vi "2021-07-09.vi"() -> ()   [LabVIEW 2019]
panel:
  out "time":cluster{i32[], i32[]}[](graph)
  out "throughput":cluster{i32[], dbl[]}[](graph)
  out "message rate":cluster{i32[], dbl[]}[](graph)
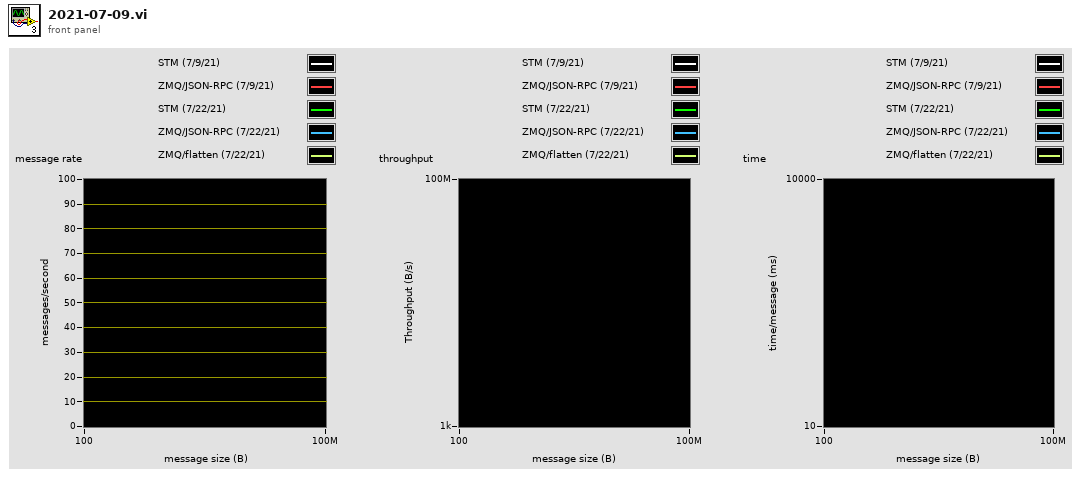
[diagram p1: front panel]
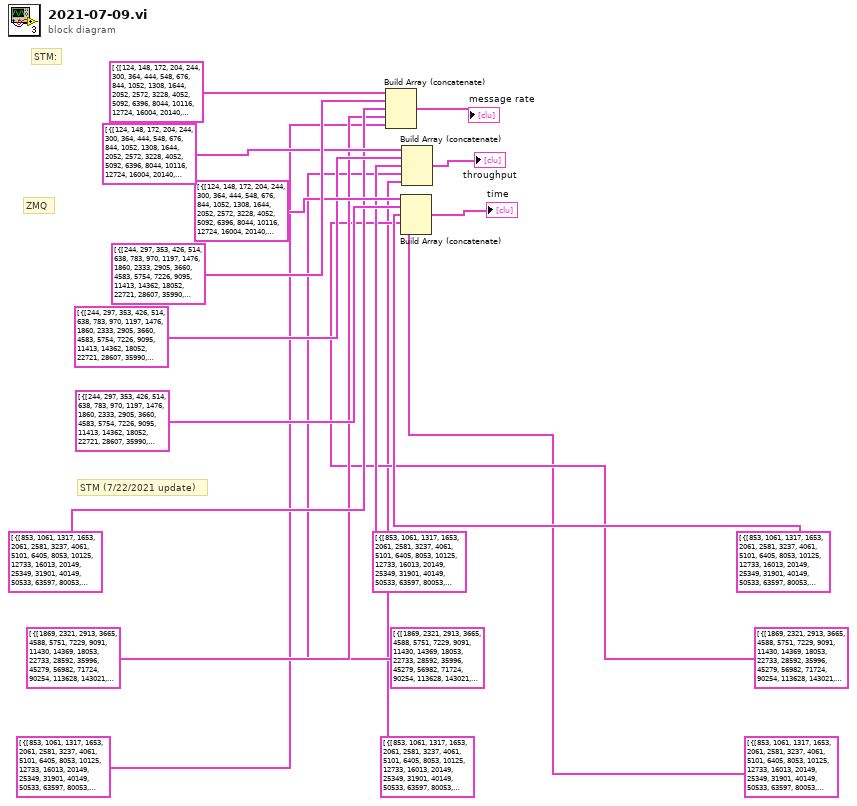
[diagram p0: block diagram]
diagram:
  # "STM (7/22/2021 update)"
  # "ZMQ"
  # "STM:"
  n1 = Build Array (concatenate)(cluster{i32[], dbl[]}[] [{[124, 148, 172, 204, 244, 300, 364, 444, 548, 676, 844, 1052, 1308, 1644, 2052, 2572, 3228, 4052, 5092, 6396, 8044, 10116, 12724, 16004, 20140, 25340, 31892, 40140, 50524, 63588, 80044, 100756, 126836, 159668, 200996, 253028, 318532, 400996, 504812, 635508, 800044, 1007188, 1267956, 1596252, 2009556, 2529868, 3184900, 4009540, 5047700, 6354668, 8000044], [73.26007326007326, 37.31343283582089, 80.32128514056225, 80.97165991902834, 83.68200836820084, 81.30081300813008, 81.30081300813008, 81.30081300813008, 80.0, 81.9672131147541, 82.3045267489712, 82.98755186721992, 81.30081300813008, 82.98755186721992, 82.3045267489712, 80.64516129032258, 80.97165991902834, 81.9672131147541, 82.64462809917356, 82.64462809917356, 81.63265306122449, 80.0, 81.9672131147541, 82.64462809917356, 78.43137254901961, 82.3045267489712, 81.30081300813008, 80.64516129032258, 80.0, 80.0, 79.6812749003984, 79.6812749003984, 79.6812749003984, 75.18796992481202, 77.22007722007721, 74.07407407407408, 71.94244604316546, 69.68641114982579, 66.22516556291392, 62.30529595015576, 57.636887608069166, 50.125313283208015, 36.03603603603603, 31.84713375796178, 27.06359945872801, 23.80952380952381, 18.099547511312217, 13.89854065323141, 9.47867298578199, 7.163323782234958, 5.396654074473826]}] ("message rate"), cluster{i32[], dbl[]}[] [{[244, 297, 353, 426, 514, 638, 783, 970, 1197, 1476, 1860, 2333, 2905, 3660, 4583, 5754, 7226, 9095, 11413, 14362, 18052, 22721, 28607, 35990, 45262, 57027, 71748, 90267, 113711, 142986, 180100, 226656, 285362, 359078, 452157, 569307, 716716, 902172, 1135653, 1430011, 1799736, 2265809, 2852633, 3591256, 4521510, 5691835, 7165085, 9020945, 11356828, 14298020, 17999563], [60.42296072507553, 60.6060606060606, 60.6060606060606, 62.5, 63.09148264984227, 58.139534883720934, 65.359477124183, 68.4931506849315, 54.200542005420054, 62.11180124223603, 60.06006006006006, 65.78947368421053, 63.291139240506325, 51.41388174807198, 63.492063492063494, 64.1025641025641, 56.81818181818182, 65.14657980456026, 56.81818181818182, 54.94505494505495, 50.76142131979695, 49.26108374384236, 50.25125628140703, 49.75124378109452, 51.0204081632653, 44.54342984409799, 42.918454935622314, 40.48582995951417, 39.920159680638726, 37.38317757009346, 32.62642740619902, 28.40909090909091, 24.96878901373283, 21.141649048625794, 18.18181818181818, 14.388489208633095, 12.453300124533001, 10.655301012253597, 8.003201280512204, 6.736274840013473, 5.442176870748299, 4.519774011299435, 3.7064492216456637, 2.983738624496494, 2.384358607534573, 1.9719976336028398, 1.5360983102918588, 1.238927089140804, 0.963762528912876, 0.7363228039172374, 0.598623166716552]}] ("message rate 2"), cluster{i32[], dbl[]}[] [{[853, 1061, 1317, 1653, 2061, 2581, 3237, 4061, 5101, 6405, 8053, 10125, 12733, 16013, 20149, 25349, 31901, 40149, 50533, 63597, 80053, 100765, 126845, 159677, 201005, 253037, 318541, 401005, 504821, 635517, 800053, 1007197, 1267965, 1596261, 2009565, 2529877, 3184909, 4009549, 5047709, 6354677, 8000053], [86.58008658008657, 87.33624454148472, 84.03361344537815, 85.47008547008546, 85.83690987124463, 85.47008547008546, 84.74576271186442, 85.83690987124463, 86.58008658008657, 86.20689655172413, 85.83690987124463, 85.1063829787234, 85.1063829787234, 84.74576271186442, 85.47008547008546, 86.20689655172413, 85.83690987124463, 85.1063829787234, 84.03361344537815, 82.3045267489712, 81.9672131147541, 82.64462809917356, 82.3045267489712, 80.64516129032258, 80.32128514056225, 79.6812749003984, 78.125, 74.07407407407408, 68.72852233676976, 69.68641114982579, 66.44518272425249, 59.347181008902076, 47.16981132075472, 39.920159680638726, 29.806259314456035, 26.52519893899204, 21.62162162162162, 16.142050040355123, 11.46131805157593, 9.7799511002445, 8.012820512820513]}] ("message rate"), cluster{i32[], dbl[]}[] [{[1869, 2321, 2913, 3665, 4588, 5751, 7229, 9091, 11430, 14369, 18053, 22733, 28592, 35996, 45279, 56982, 71724, 90254, 113628, 143021, 179910, 226633, 285458, 359226, 452070, 569242, 716757, 902238, 1135863, 1429968, 1799833, 2266041, 2852441, 3591671, 4520575, 5692223], [48.07692307692308, 95.23809523809524, 82.98755186721992, 88.88888888888889, 86.58008658008657, 81.63265306122449, 81.30081300813008, 79.05138339920948, 78.74015748031496, 74.9063670411985, 72.46376811594202, 70.92198581560284, 68.25938566552901, 64.72491909385113, 59.52380952380952, 56.980056980056986, 52.770448548812666, 45.04504504504504, 55.71030640668524, 42.19409282700422, 30.627871362940276, 32.520325203252035, 24.301336573511545, 19.821605550049554, 17.574692442882252, 13.812154696132596, 11.031439602868174, 8.92458723784025, 6.715916722632639, 5.303632988597189, 4.039587962027873, 3.2997855139415937, 2.839698991906858, 2.18435998252512, 1.7462673535318258, 1.3844662882458811]}] ("message rate"), cluster{i32[], dbl[]}[] [{[853, 1061, 1317, 1653, 2061, 2581, 3237, 4061, 5101, 6405, 8053, 10125, 12733, 16013, 20149, 25349, 31901, 40149, 50533, 63597, 80053, 100765, 126845, 159677, 201005, 253037, 318541, 401005, 504821, 635517, 800053, 1007197, 1267965, 1596261, 2009565, 2529877, 3184909, 4009549, 5047709, 6354677, 8000053], [78.125, 79.6812749003984, 77.82101167315174, 78.74015748031496, 81.30081300813008, 79.6812749003984, 79.6812749003984, 79.05138339920948, 79.36507936507937, 80.0, 77.82101167315174, 80.0, 79.05138339920948, 78.74015748031496, 80.0, 79.6812749003984, 78.125, 78.125, 78.43137254901961, 78.125, 77.22007722007721, 76.33587786259541, 76.62835249042145, 76.04562737642586, 72.992700729927, 71.17437722419928, 67.79661016949153, 64.72491909385113, 59.88023952095808, 56.17977528089888, 50.63291139240506, 43.47826086956522, 30.2571860816944, 26.917900403768506, 22.988505747126435, 20.876826722338205, 17.74622892635315, 14.673514306676449, 11.641443538998836, 9.775171065493646, 7.760962359332558]}] ("message rate")) -> (→"message rate":cluster{i32[], dbl[]}[])
  n2 = Build Array (concatenate)(cluster{i32[], i32[]}[] [{[124, 148, 172, 204, 244, 300, 364, 444, 548, 676, 844, 1052, 1308, 1644, 2052, 2572, 3228, 4052, 5092, 6396, 8044, 10116, 12724, 16004, 20140, 25340, 31892, 40140, 50524, 63588, 80044, 100756, 126836, 159668, 200996, 253028, 318532, 400996, 504812, 635508, 800044, 1007188, 1267956, 1596252, 2009556, 2529868, 3184900, 4009540, 5047700, 6354668, 8000044], [14, 27, 12, 12, 12, 12, 12, 12, 12, 12, 12, 12, 12, 12, 12, 12, 12, 12, 12, 12, 12, 12, 12, 12, 13, 12, 12, 12, 12, 12, 13, 13, 13, 13, 13, 14, 14, 14, 15, 16, 17, 19, 27, 31, 36, 41, 54, 71, 104, 138, 183]}] ("time"), cluster{i32[], i32[]}[] [{[244, 297, 353, 426, 514, 638, 783, 970, 1197, 1476, 1860, 2333, 2905, 3660, 4583, 5754, 7226, 9095, 11413, 14362, 18052, 22721, 28607, 35990, 45262, 57027, 71748, 90267, 113711, 142986, 180100, 226656, 285362, 359078, 452157, 569307, 716716, 902172, 1135653, 1430011, 1799736, 2265809, 2852633, 3591256, 4521510, 5691835, 7165085, 9020945, 11356828, 14298020, 17999563], [17, 16, 16, 16, 16, 17, 15, 15, 18, 16, 17, 15, 16, 19, 16, 16, 18, 15, 18, 18, 20, 20, 20, 20, 20, 22, 23, 25, 25, 27, 31, 35, 40, 47, 55, 70, 80, 94, 125, 148, 183, 221, 269, 335, 418, 506, 650, 805, 1035, 1355, 1666]}] ("time 2"), cluster{i32[], i32[]}[] [{[853, 1061, 1317, 1653, 2061, 2581, 3237, 4061, 5101, 6405, 8053, 10125, 12733, 16013, 20149, 25349, 31901, 40149, 50533, 63597, 80053, 100765, 126845, 159677, 201005, 253037, 318541, 401005, 504821, 635517, 800053, 1007197, 1267965, 1596261, 2009565, 2529877, 3184909, 4009549, 5047709, 6354677, 8000053], [12, 11, 12, 12, 12, 12, 12, 12, 11, 12, 12, 12, 12, 12, 12, 12, 12, 12, 12, 12, 12, 12, 12, 12, 12, 12, 12, 13, 14, 14, 14, 16, 20, 24, 32, 36, 44, 58, 83, 97, 119]}] ("time"), cluster{i32[], i32[]}[] [{[1869, 2321, 2913, 3665, 4588, 5751, 7229, 9091, 11430, 14369, 18053, 22733, 28592, 35996, 45279, 56982, 71724, 90254, 113628, 143021, 179910, 226633, 285458, 359226, 452070, 569242, 716757, 902238, 1135863, 1429968, 1799833, 2266041, 2852441, 3591671, 4520575, 5692223], [21, 10, 12, 11, 12, 12, 12, 13, 13, 13, 14, 14, 15, 15, 17, 18, 19, 22, 18, 24, 33, 31, 41, 50, 57, 72, 90, 112, 149, 188, 247, 302, 351, 457, 572, 721]}] ("time"), cluster{i32[], i32[]}[] [{[853, 1061, 1317, 1653, 2061, 2581, 3237, 4061, 5101, 6405, 8053, 10125, 12733, 16013, 20149, 25349, 31901, 40149, 50533, 63597, 80053, 100765, 126845, 159677, 201005, 253037, 318541, 401005, 504821, 635517, 800053, 1007197, 1267965, 1596261, 2009565, 2529877, 3184909, 4009549, 5047709, 6354677, 8000053], [13, 12, 13, 13, 12, 13, 13, 13, 13, 12, 13, 12, 13, 13, 12, 12, 13, 13, 13, 13, 13, 13, 13, 13, 13, 14, 14, 15, 16, 17, 19, 22, 32, 36, 42, 46, 54, 65, 82, 98, 122]}] ("time")) -> (→"time":cluster{i32[], i32[]}[])
  n3 = Build Array (concatenate)(cluster{i32[], dbl[]}[] [{[124, 148, 172, 204, 244, 300, 364, 444, 548, 676, 844, 1052, 1308, 1644, 2052, 2572, 3228, 4052, 5092, 6396, 8044, 10116, 12724, 16004, 20140, 25340, 31892, 40140, 50524, 63588, 80044, 100756, 126836, 159668, 200996, 253028, 318532, 400996, 504812, 635508, 800044, 1007188, 1267956, 1596252, 2009556, 2529868, 3184900, 4009540, 5047700, 6354668, 8000044], [9084.249084249084, 5522.388059701492, 13815.261044176706, 16518.218623481782, 20418.410041841005, 24390.243902439026, 29593.49593495935, 36097.560975609755, 43840.0, 55409.83606557377, 69465.02057613169, 87302.90456431535, 106341.46341463414, 136431.53526970954, 168888.8888888889, 207419.35483870967, 261376.51821862347, 332131.1475409836, 420826.4462809918, 528595.0413223141, 656653.0612244898, 809280.0, 1042950.8196721312, 1322644.6280991735, 1579607.843137255, 2085596.70781893, 2592845.5284552844, 3237096.7741935486, 4041920.0, 5087040.0, 6378007.96812749, 8028366.533864542, 10106454.183266932, 12005112.781954886, 15520926.64092664, 18742814.814814813, 22915971.22302158, 27943972.125435542, 33431258.278145697, 39595514.018691584, 46112046.10951009, 50485614.03508772, 45692108.1081081, 50836050.95541401, 54385818.673883624, 60234952.38095238, 57645248.86877828, 55726754.69075747, 47845497.630331755, 45520544.412607454, 43173470.04856989]}] ("throughput"), cluster{i32[], dbl[]}[] [{[244, 297, 353, 426, 514, 638, 783, 970, 1197, 1476, 1860, 2333, 2905, 3660, 4583, 5754, 7226, 9095, 11413, 14362, 18052, 22721, 28607, 35990, 45262, 57027, 71748, 90267, 113711, 142986, 180100, 226656, 285362, 359078, 452157, 569307, 716716, 902172, 1135653, 1430011, 1799736, 2265809, 2852633, 3591256, 4521510, 5691835, 7165085, 9020945, 11356828, 14298020, 17999563], [14743.202416918428, 18000.0, 21393.939393939392, 26625.0, 32429.022082018928, 37093.023255813954, 51176.470588235294, 66438.35616438357, 64878.04878048781, 91677.01863354037, 111711.7117117117, 153486.84210526317, 183860.7594936709, 188174.80719794345, 290984.126984127, 368846.1538461539, 410568.1818181818, 592508.1433224756, 648465.9090909092, 789120.8791208791, 916345.1776649746, 1119261.0837438423, 1437537.688442211, 1790547.263681592, 2309285.714285714, 2540178.1737193763, 3079313.30472103, 3654534.4129554657, 4539361.27744511, 5345271.028037383, 5876019.5758564435, 6439090.909090909, 7125143.570536829, 7591501.057082453, 8221036.363636363, 8191467.625899281, 8925479.452054795, 9612914.224826852, 9088859.543817526, 9632947.120242506, 9794481.632653061, 10240944.632768363, 10573139.362490734, 10715369.237654781, 10780901.287553648, 11224285.15085782, 11006274.961597543, 11176293.13014929, 10945285.27370856, 10527958.176864738, 10774955.402574081]}] ("throughput 2"), cluster{i32[], dbl[]}[] [{[853, 1061, 1317, 1653, 2061, 2581, 3237, 4061, 5101, 6405, 8053, 10125, 12733, 16013, 20149, 25349, 31901, 40149, 50533, 63597, 80053, 100765, 126845, 159677, 201005, 253037, 318541, 401005, 504821, 635517, 800053, 1007197, 1267965, 1596261, 2009565, 2529877, 3184909, 4009549, 5047709, 6354677, 8000053], [73852.81385281385, 92663.75545851528, 110672.26890756303, 141282.05128205128, 176909.87124463517, 220598.2905982906, 274322.0338983051, 348583.69098712446, 441645.0216450216, 552155.172413793, 691244.635193133, 861702.1276595745, 1083659.574468085, 1357033.8983050848, 1722136.752136752, 2185258.620689655, 2738283.261802575, 3416936.170212766, 4246470.588235294, 5234320.987654321, 6561721.31147541, 8327685.950413223, 10439917.695473252, 12877177.41935484, 16144979.919678714, 20162310.75697211, 24886015.625, 29704074.07407407, 34695601.37457045, 44286898.95470384, 53159667.77408638, 59774302.67062314, 59809669.81132076, 63722994.01197605, 59897615.49925484, 67105490.71618037, 68862897.2972973, 64722340.59725585, 57853398.28080229, 62148430.317848414, 64102988.78205128]}] ("throughput"), cluster{i32[], dbl[]}[] [{[1869, 2321, 2913, 3665, 4588, 5751, 7229, 9091, 11430, 14369, 18053, 22733, 28592, 35996, 45279, 56982, 71724, 90254, 113628, 143021, 179910, 226633, 285458, 359226, 452070, 569242, 716757, 902238, 1135863, 1429968, 1799833, 2266041, 2852441, 3591671, 4520575, 5692223], [89855.76923076923, 221047.61904761905, 241742.73858921163, 325777.77777777775, 397229.43722943723, 469469.38775510207, 587723.5772357724, 718656.1264822134, 900000.0, 1076329.5880149812, 1308188.4057971013, 1612269.5035460994, 1951672.3549488056, 2329838.1877022656, 2695178.5714285714, 3246837.606837607, 3784907.6517150397, 4065495.4954954954, 6330250.69637883, 6034641.350210971, 5510260.336906585, 7370178.861788618, 6937010.935601459, 7120436.075322102, 7944991.212653779, 7862458.563535912, 7906861.555432985, 8052101.740294511, 7628361.316319677, 7584025.457438345, 7270583.720460514, 7477449.265797723, 8100073.83217379, 7845502.402795981, 7894132.541692133, 7880690.8486778345]}] ("throughput"), cluster{i32[], dbl[]}[] [{[853, 1061, 1317, 1653, 2061, 2581, 3237, 4061, 5101, 6405, 8053, 10125, 12733, 16013, 20149, 25349, 31901, 40149, 50533, 63597, 80053, 100765, 126845, 159677, 201005, 253037, 318541, 401005, 504821, 635517, 800053, 1007197, 1267965, 1596261, 2009565, 2529877, 3184909, 4009549, 5047709, 6354677, 8000053], [66640.625, 84541.83266932271, 102490.27237354085, 130157.48031496063, 167560.9756097561, 205657.3705179283, 257928.28685258963, 321027.6679841897, 404841.2698412698, 512400.0, 626692.607003891, 810000.0, 1006561.2648221344, 1260866.1417322834, 1611920.0, 2019840.637450199, 2492265.625, 3136640.625, 3963372.5490196077, 4968515.625, 6181698.841698841, 7691984.732824427, 9719923.371647509, 12142737.642585551, 14671897.810218977, 18009750.889679715, 21596000.0, 25955016.181229774, 30228802.39520958, 35703202.24719101, 40509012.658227846, 43791173.91304348, 38365052.95007564, 42967994.61641992, 46196896.551724136, 52815803.75782881, 56520124.22360248, 58834174.61482025, 58762619.324796274, 62118054.740957975, 62088110.20566551]}] ("throughput")) -> (→"throughput":cluster{i32[], dbl[]}[])
